vi "test unknown resource.vi"(8 "error in (no error)":errorcluster) -> (0 "error out":errorcluster, 3 "body":string)   [LabVIEW 2020, in "MCP Server tests.lvlib"]
doc: "resources/read for a uri that does not exist must be answered with a JSON-RPC error object (code -32002, a message) that carries the id of the request. The LabVIEW error cluster (status, source) must not appear in the answer."
uses:
  MCP Server tests.lvlib
  <vilib>/JDP Science/JSONtext/Next JSON Value.vi
  <vilib>/JDP Science/JSONtext/String Subset.vi
  <vilib>/JDP Science/JSONtext/Parsing/Advance past next JSON Value (inlined COPY).vi
  <vilib>/JDP Science/JSONtext/Parsing/Advance past whitespace.vi
  <vilib>/JDP Science/JSONtext/Parsing/Advance past String.vi
  <vilib>/JDP Science/JSONtext/Parsing/Advance past Number.vi
  <vilib>/JDP Science/JSONtext/Parsing/Advance past Line Ending.vi
  <vilib>/JDP Science/JSONtext/Parsing/Parse Full Path or Item Name.vi
  <vilib>/JDP Science/JSONtext/Parsing/Advance past Array.vi
  <vilib>/JDP Science/JSONtext/Parsing/Advance past Object.vi
  <vilib>/JDP Science/JSONtext/support/Error Cluster From Code.vi
  <vilib>/JDP Science/JSONtext/Offset/Find Item Locations by Path.vi
  <vilib>/addons/_JKI Toolkits/Caraya/classes/Test/Test.lvclass
  <vilib>/JDP Science/JSONtext/JSONtext.lvlib
  <vilib>/addons/_JKI Toolkits/Caraya/classes/Assert/Assert.lvclass
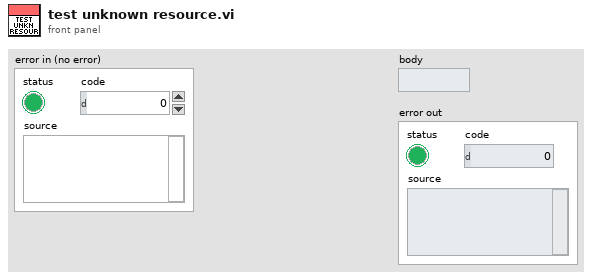
[diagram p1: front panel]
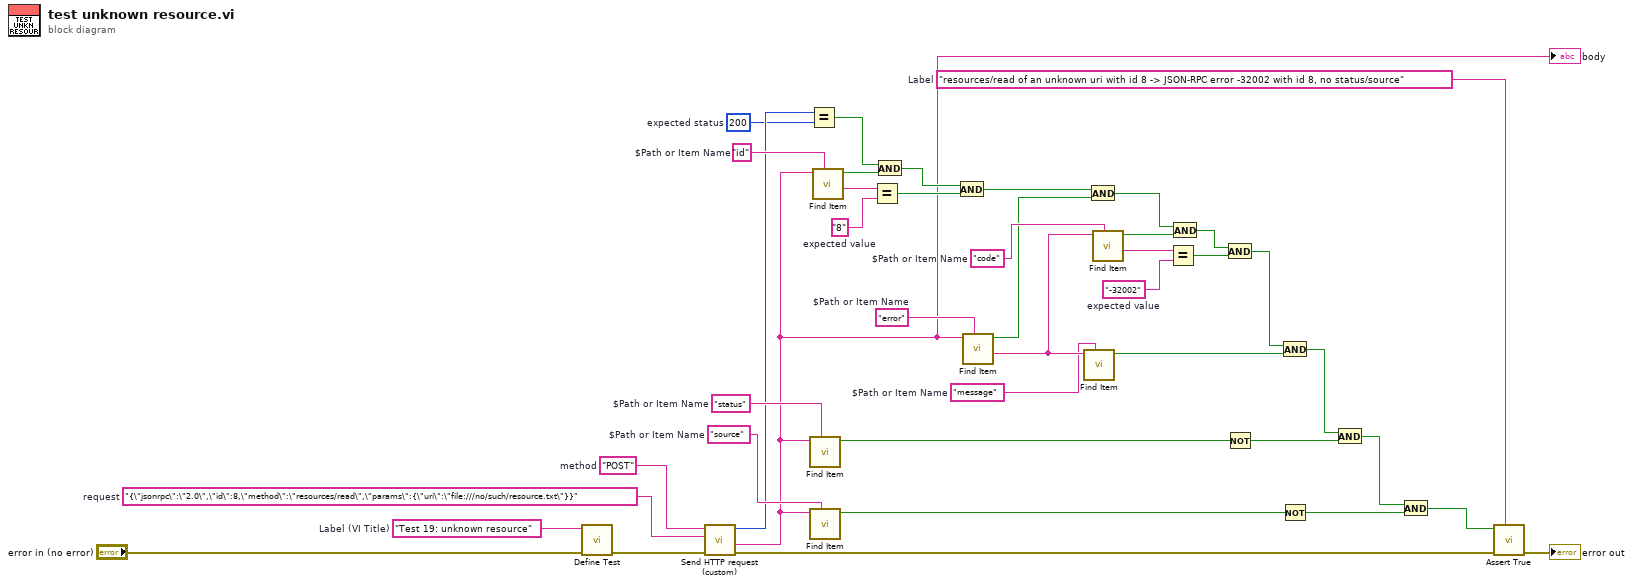
[diagram p0: block diagram]
diagram:
  w3 = "resources/read of an unknown uri with id 8 -> JSON-RPC error -32002 with id 8, no status/source"  # Label
  w24 = "-32002"  # expected value
  w26 = "8"  # expected value
  w28 = 200  # expected status
  w30 = "source"  # $Path or Item Name
  w31 = "status"  # $Path or Item Name
  w32 = "message"  # $Path or Item Name
  w34 = "code"  # $Path or Item Name
  w35 = "error"  # $Path or Item Name
  w36 = "id"  # $Path or Item Name
  w38 = "{\"jsonrpc\":\"2.0\",\"id\":8,\"method\":\"resources/read\",\"params\":{\"uri\":\"file:///no/such/resource.txt\"}}"  # request
  w39 = "POST"  # method
  w41 = "Test 19: unknown resource"  # Label (VI Title)
  n1 = call <vilib>:"Define Test.vi"("error in (no error)"="error in (no error)", "Label (VI Title)"=w41) -> ("error out"=w37:errorcluster)  [unwired: 8 in, 1 out]
  n2 = call "Send HTTP request (custom).vi"("error in (no error)"=w37, "request"=w38, "method"=w39) -> ("error out"=w4:errorcluster, "response"=w2:string, "status code"=w29:i32)  [unwired: 5 in, 1 out]
  "body" <- w2
  n3 = Equal?(x=w29, y=w28) -> (x = y?=w21:bool)
  n4 = call <vilib>:"Find Item.vi"("$Path or Item Name"=w31, "JSON"=w2) -> ("Found"=w23:bool)  [unwired: 6 in, 3 out]
  n5 = call <vilib>:"Find Item.vi"("$Path or Item Name"=w30, "JSON"=w2) -> ("Found"=w22:bool)  [unwired: 6 in, 3 out]
  n6 = call <vilib>:"Find Item.vi"("$Path or Item Name"=w36, "JSON"=w2) -> ("<JSON>"=w27:string, "Found"=w20:bool)  [unwired: 6 in, 2 out]
  n7 = Equal?(x=w27, y=w26) -> (x = y?=w18:bool)
  n8 = And(x=w21, y=w20) -> (x .and. y?=w19:bool)
  n9 = And(x=w19, y=w18) -> (x .and. y?=w17:bool)
  n10 = call <vilib>:"Find Item.vi"("$Path or Item Name"=w35, "JSON"=w2) -> ("<JSON>"=w33:string, "Found"=w16:bool)  [unwired: 6 in, 2 out]
  n11 = call <vilib>:"Find Item.vi"("$Path or Item Name"=w32, "JSON"=w33) -> ("Found"=w10:bool)  [unwired: 6 in, 3 out]
  n12 = And(x=w17, y=w16) -> (x .and. y?=w15:bool)
  n13 = call <vilib>:"Find Item.vi"("$Path or Item Name"=w34, "JSON"=w33) -> ("<JSON>"=w25:string, "Found"=w14:bool)  [unwired: 6 in, 2 out]
  n14 = Equal?(x=w25, y=w24) -> (x = y?=w12:bool)
  n15 = And(x=w15, y=w14) -> (x .and. y?=w13:bool)
  n16 = And(x=w13, y=w12) -> (x .and. y?=w11:bool)
  n17 = Not(x=w23) -> (.not. x?=w8:bool)
  n18 = And(x=w11, y=w10) -> (x .and. y?=w9:bool)
  n19 = Not(x=w22) -> (.not. x?=w6:bool)
  n20 = And(x=w9, y=w8) -> (x .and. y?=w7:bool)
  n21 = And(x=w7, y=w6) -> (x .and. y?=w5:bool)
  n22 = call <vilib>:"Assert True.vi"("Label"=w3, "error in (no error)"=w4, "True?"=w5) -> ("error out"=→"error out":errorcluster)  [unwired: 7 in, 1 out]
